vi "test Get-Set-Get Default Word Value.vi"(8 "error in":errorcluster, 11 "TestCase in":refnum<class "Scripting.lvclass">) -> (0 "error out":errorcluster, 3 "TestCase out":refnum<class "Scripting.lvclass">)   [LabVIEW 2020, in "Scripting.lvclass"]
uses:
  Scripting.lvclass
  <vilib>/addons/_JKI Toolkits/VI Tester/TestCase.llb/TestCase.lvclass
  Scripting/AIM/AIM ARINC 429 Scripting.lvlib
  <vilib>/NI/NI VeriStand Encoding and Decoding/Encoding.ctl
  <vilib>/NI/NI VeriStand Encoding and Decoding/Encoding and Decoding.lvlib
  Shared/Parameter Definition.ctl
  Shared/VS Channel Definition for Parameter.ctl
  Shared/Transfer Type.ctl
  Shared/VS Channels Definition for Label.ctl
  Shared/Direction.ctl
  Shared/Transfer Speed.ctl
  C:/Program Files (x86)/National Instruments/LabVIEW 2020/vi.lib/addons/_JKI Toolkits/VI Tester/TestCase.llb/TestCase.lvclass
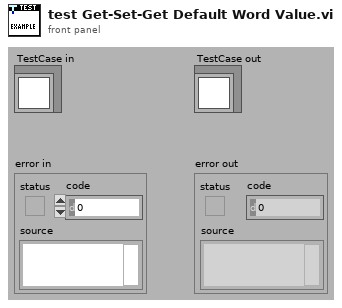
[diagram p1: front panel]
types:
  T1 = typedef "Transfer Speed.ctl" = enum16{"LO (12.5 kb/s)", "HI (100 kb/s)"}
  T2 = typedef "Direction.ctl" = enum16{"Rx", "Tx"}
  T3 = typedef "VS Channels Definition for Label.ctl" = cluster{"label (Dec)":u32, "parameters":T4[], "SDI value":u8, "SDI enabled":bool, "transfer type":T7, "create timestamp":bool, "transmit period":u32}
  T4 = typedef "VS Channel Definition for Parameter.ctl" = cluster{"name":string, "unit":string, "Parameter":T5}
  T5 = typedef "Parameter Definition.ctl" = cluster{"start index":i32, "size":i32, "encoding":T6, "signed":bool, "scale multiplier":dbl, "scale offset":dbl, "default value":dbl}
  T6 = typedef "Encoding and Decoding.lvlib/Encoding.ctl" = enum16{"BNR", "BCD", "Discrete"}
  T7 = typedef "Transfer Type.ctl" = enum16{"Scheduled", "Acyclic", "Block", "Strobe"}
  T8 = typedef "Custom Device API.lvlib/Custom Device Item Ref.ctl" = u64
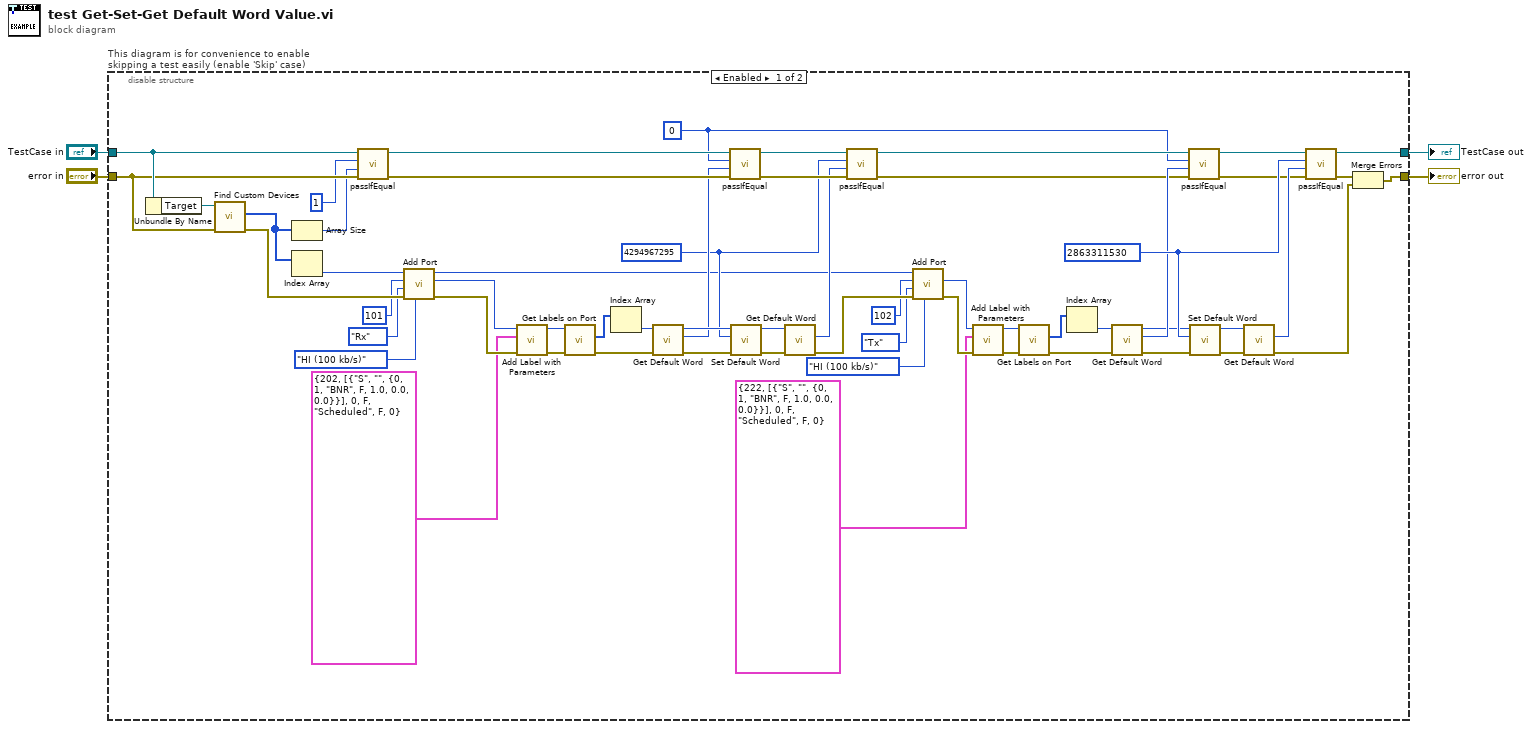
[diagram p0: block diagram]
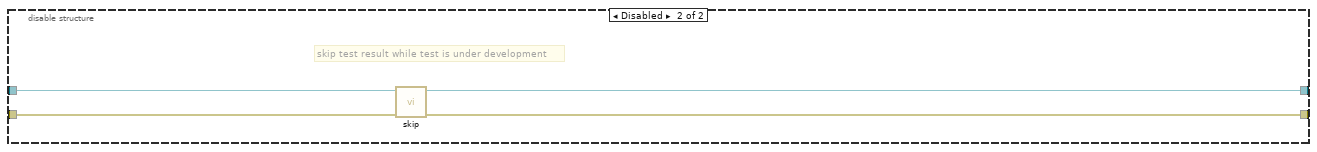
[diagram p2: hidden frame]
diagram:
  n1 = disable-structure "This diagram is for convenience to enable skipping a test easily (enable 'Skip' case)" shown="Enabled" {
    disable-tunnel: "TestCase in" -> [w62 w67]
    disable-tunnel: [w27 w65] -> w1
    disable-tunnel: [w58 w66] -> w3
    disable-tunnel: "error in" -> [w61 w64]
    frame Enabled {
      w41 = u32 2863311530 ("default word")
      w44 = u32 4294967295 ("default word")
      w26 = u32 0 ("default word")
      n2 = Unbundle By Name(w62) -> ("Target"=w63:refnum<k24>)
      n3 = call "Find Custom Devices.vi"("error in"=w61, "target in"=w63) -> ("error out"=w23:errorcluster, "AIM ARINC 429 custom devices"=w25:u64[])  [unwired: 7 in, 1 out]
      n4 = Array Size(array=w25) -> (size(s)=w59:i32)
      n5 = Index Array(array=w25) -> (element=w24:u64)  [unwired: 1 in]
      n6 = call-dynamic "passIfEqual.vi"("error in (no error)"=w61, "y"=w59, "x"=1 ("size(s)"), "TestCase in"=w62) -> ("error out"=w48:errorcluster, "TestCase out"=w49:refnum<class "Scripting.lvclass">)  [unwired: 6 in]
      n7 = call "Add Port.vi"("speed"=Transfer_Speed."HI (100 kb/s)", "error in"=w23, "direction"=Direction."Rx", "port number"=u16 101, "AIM ARINC 429 custom device in"=w24) -> ("error out"=w17:errorcluster, "port"=w18:T8, "AIM ARINC 429 custom device out"=w21:T8)  [unwired: 4 in]
      n8 = call "Add Label with Parameters.vi"("error in"=w17, "label"=T3 {"label (Dec)"=202, "parameters"=[{"name"="S", "unit"="", "Parameter"={"start index"=0, "size"=1, "encoding"=enum."BNR", "signed"=FALSE, "scale multiplier"=1.0, "scale offset"=0.0, "default value"=0.0}}], "SDI value"=0, "SDI enabled"=FALSE, "transfer type"=enum."Scheduled", "create timestamp"=FALSE, "transmit period"=0}, "port ref"=w18) -> ("error out"=w15:errorcluster, "port ref out"=w14:T8)  [unwired: 7 in]
      n9 = call "Get Labels on Port.vi"("error in"=w15, "port in"=w14) -> ("error out"=w55:errorcluster, "labels"=w56:T8[])  [unwired: 6 in, 2 out]
      n10 = Index Array(array=w56) -> (element=w54:T8)  [unwired: 1 in]
      n11 = call "Get Default Word.vi"("error in"=w55, "Item Ref in"=w54) -> ("error out"=w53:errorcluster, "default word"=w47:u32, "Item Ref out"=w52:T8)  [unwired: 7 in]
      n12 = call-dynamic "passIfEqual.vi"("error in (no error)"=w48, "y"=w47, "x"=w26, "TestCase in"=w49) -> ("error out"=w45:errorcluster, "TestCase out"=w46:refnum<class "Scripting.lvclass">)  [unwired: 6 in]
      n13 = call "Set Default Word.vi"("error in"=w53, "default word"=w44, "label ref in"=w52) -> ("error out"=w51:errorcluster, "label ref out"=w50:T8)  [unwired: 7 in]
      n14 = call "Get Default Word.vi"("error in"=w51, "Item Ref in"=w50) -> ("error out"=w20:errorcluster, "default word"=w43:u32)  [unwired: 7 in, 1 out]
      n15 = call-dynamic "passIfEqual.vi"("error in (no error)"=w45, "y"=w43, "x"=w44, "TestCase in"=w46) -> ("error out"=w34:errorcluster, "TestCase out"=w30:refnum<class "Scripting.lvclass">)  [unwired: 6 in]
      n16 = call "Add Port.vi"("speed"=Transfer_Speed."HI (100 kb/s)", "error in"=w20, "direction"=Direction."Tx", "port number"=u16 102, "AIM ARINC 429 custom device in"=w21) -> ("error out"=w12:errorcluster, "port"=w13:T8)  [unwired: 4 in, 1 out]
      n17 = call "Add Label with Parameters.vi"("error in"=w12, "label"=T3 {"label (Dec)"=222, "parameters"=[{"name"="S", "unit"="", "Parameter"={"start index"=0, "size"=1, "encoding"=enum."BNR", "signed"=FALSE, "scale multiplier"=1.0, "scale offset"=0.0, "default value"=0.0}}], "SDI value"=0, "SDI enabled"=FALSE, "transfer type"=enum."Scheduled", "create timestamp"=FALSE, "transmit period"=0}, "port ref"=w13) -> ("error out"=w10:errorcluster, "port ref out"=w11:T8)  [unwired: 7 in]
      n18 = call "Get Labels on Port.vi"("error in"=w10, "port in"=w11) -> ("error out"=w33:errorcluster, "labels"=w57:T8[])  [unwired: 6 in, 2 out]
      n19 = Index Array(array=w57) -> (element=w32:T8)  [unwired: 1 in]
      n20 = call "Get Default Word.vi"("error in"=w33, "Item Ref in"=w32) -> ("error out"=w35:errorcluster, "default word"=w39:u32, "Item Ref out"=w36:T8)  [unwired: 7 in]
      n21 = call-dynamic "passIfEqual.vi"("error in (no error)"=w34, "y"=w39, "x"=w26, "TestCase in"=w30) -> ("error out"=w40:errorcluster, "TestCase out"=w29:refnum<class "Scripting.lvclass">)  [unwired: 6 in]
      n22 = call "Set Default Word.vi"("error in"=w35, "default word"=w41, "label ref in"=w36) -> ("error out"=w37:errorcluster, "label ref out"=w38:T8)  [unwired: 7 in]
      n23 = call "Get Default Word.vi"("error in"=w37, "Item Ref in"=w38) -> ("error out"=w31:errorcluster, "default word"=w42:u32)  [unwired: 7 in, 1 out]
      n24 = call-dynamic "passIfEqual.vi"("error in (no error)"=w40, "y"=w42, "x"=w41, "TestCase in"=w29) -> ("error out"=w28:errorcluster, "TestCase out"=w27:refnum<class "Scripting.lvclass">)  [unwired: 6 in]
      n25 = Merge Errors(w28, w31) -> (w58:errorcluster)
    }
    frame Disabled {
      # "skip test result while test is under development"
      n26 = call <vilib>:"skip.vi"("error in (no error)"=w64, "TestCase in"=w67) -> ("error out"=w66:errorcluster, "TestCase out"=w65:refnum<class "Scripting.lvclass">)  [unwired: 8 in]
    }
  }
  "error out" <- w3
  "TestCase out" <- w1
